vi "Plugin_Editor.vi"(8 "error in (no error)":errorcluster={"status"=FALSE, "code"=0, "source"="\"\""}, 10 "target inventory":string, 11 "PluginManifest":string) -> (0 "error out":errorcluster={"status"=FALSE, "code"=0, "source"="\"\""}, 2 "status ok":bool, 3 "Selected plugin definitions":string)   [LabVIEW 2026]
doc: "INTENT: Register supported custom VIs. LOGIC: Show plugin ID/version, target support, arguments, outputs, resource requirements and cancellation policy."
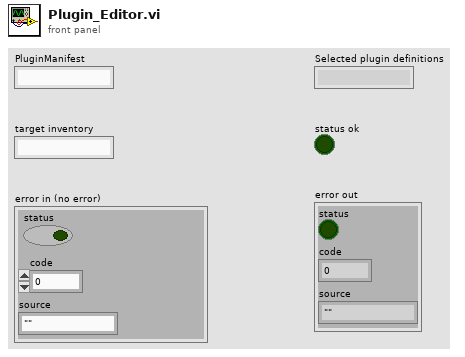
[diagram p1: front panel]
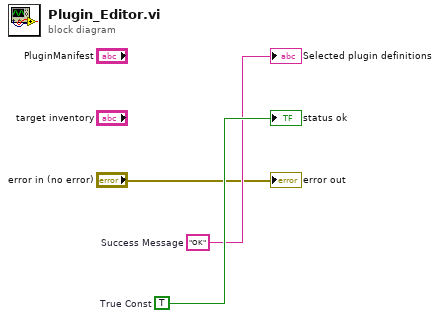
[diagram p0: block diagram]
diagram:
  w3 = TRUE  # True Const
  w2 = "OK"  # Success Message
  "Selected plugin definitions" <- w2
  "status ok" <- w3
  "error out" <- "error in (no error)"
